vi "Drive Controller.vi"(8 "error in":errorcluster) -> ()   [LabVIEW 2025]
doc: "This VI executes continuously carrying out the current operation and responding to updates or new operation requests. It will often contain the timing or control code that is difficult to place directly in TeleOp. This VI generally opens all sensors and motors and isolates the rest of the robot code from knowing implementation details of how the operations are carried out."
uses:
  <vilib>/Rock Robotics/WPI/Framework/Completion Status.ctl
  Drive Setpoints.ctl
  Drive Operations.ctl
  bordeaux-main/Bordeaux/Types/Single Cmd Info.ctl
  <vilib>/picture/picture.llb/imagedata.ctl
  bordeaux-main/Bordeaux/Types/Trajectory Data.ctl
  bordeaux-main/Bordeaux/Types/Segment Type.ctl
  <vilib>/Rock Robotics/WPI/ThirdParty/REV Robotics/REVLib/Typedef/SPARK PID Gains.ctl
  <vilib>/Rock Robotics/WPI/ThirdParty/REV Robotics/REVLib/Typedef/SPARK Feed Forward Gains.ctl
  <vilib>/Rock Robotics/WPI/ThirdParty/REV Robotics/REVLib/Typedef/Spark MAX Idle Mode.ctl
  <vilib>/Rock Robotics/WPI/ThirdParty/REV Robotics/REVLib/Typedef/Spark MAX Control Type.ctl
  <vilib>/Rock Robotics/WPI/ThirdParty/REV Robotics/REVLib/SubVI/Public/SPARK Open Brushless.vi
  <vilib>/Rock Robotics/WPI/ThirdParty/REV Robotics/REVLib/SubVI/Public/SPARK Configure Power Current Limit.vi
  <vilib>/Rock Robotics/WPI/ThirdParty/REV Robotics/REVLib/SubVI/Public/SPARK Configure Follower Mode From Ref.vi
  <vilib>/Rock Robotics/WPI/ThirdParty/REV Robotics/REVLib/SubVI/Public/SPARK Configure Basic Idle Mode.vi
  <vilib>/Rock Robotics/WPI/ThirdParty/REV Robotics/REVLib/SubVI/Public/SPARK Configure Closed Loop Gains.vi
  <vilib>/Rock Robotics/WPI/ThirdParty/REV Robotics/REVLib/SubVI/Public/SPARK Get Encoder Status Velocity.vi
panel:
  out "Right Motors":cluster{"Sensor Velocity":dbl, dbl}(graph)={"Sensor Velocity"=-0.0, 428.5718688964844}
  out "Left Motors":cluster{dbl, "Sensor Velocity":dbl}(graph)={0.0, "Sensor Velocity"=337.14349365234375}
  in  "Feed Forward Gains":T1={"kV"=0.0022, "kS"=0.0, "kA"=0.0, "kG"=0.0, "kCos"=0.0, "kCosRatio"=0.0}
  in  "PID Gains":T2={"kP"=0.0003, "kI"=0.0, "kD"=0.0}
  in  "V Scale":dbl=1.0
  in  "Interactive Values":T3
  in  "Buttons":cluster{"Execute Cmd":bool, "Abort Cmd":bool}
  out "Command Timing":cluster{"Start Time (ms)":u32, "Iterations":i32}
  out "Status":T9
  out "Current\nCmd":string
  # "Interactive Command: You may fill in the settings for a command\nand schedule it with the Execute button. You can observe and abort\nany command while fine tuning the code for the controller."
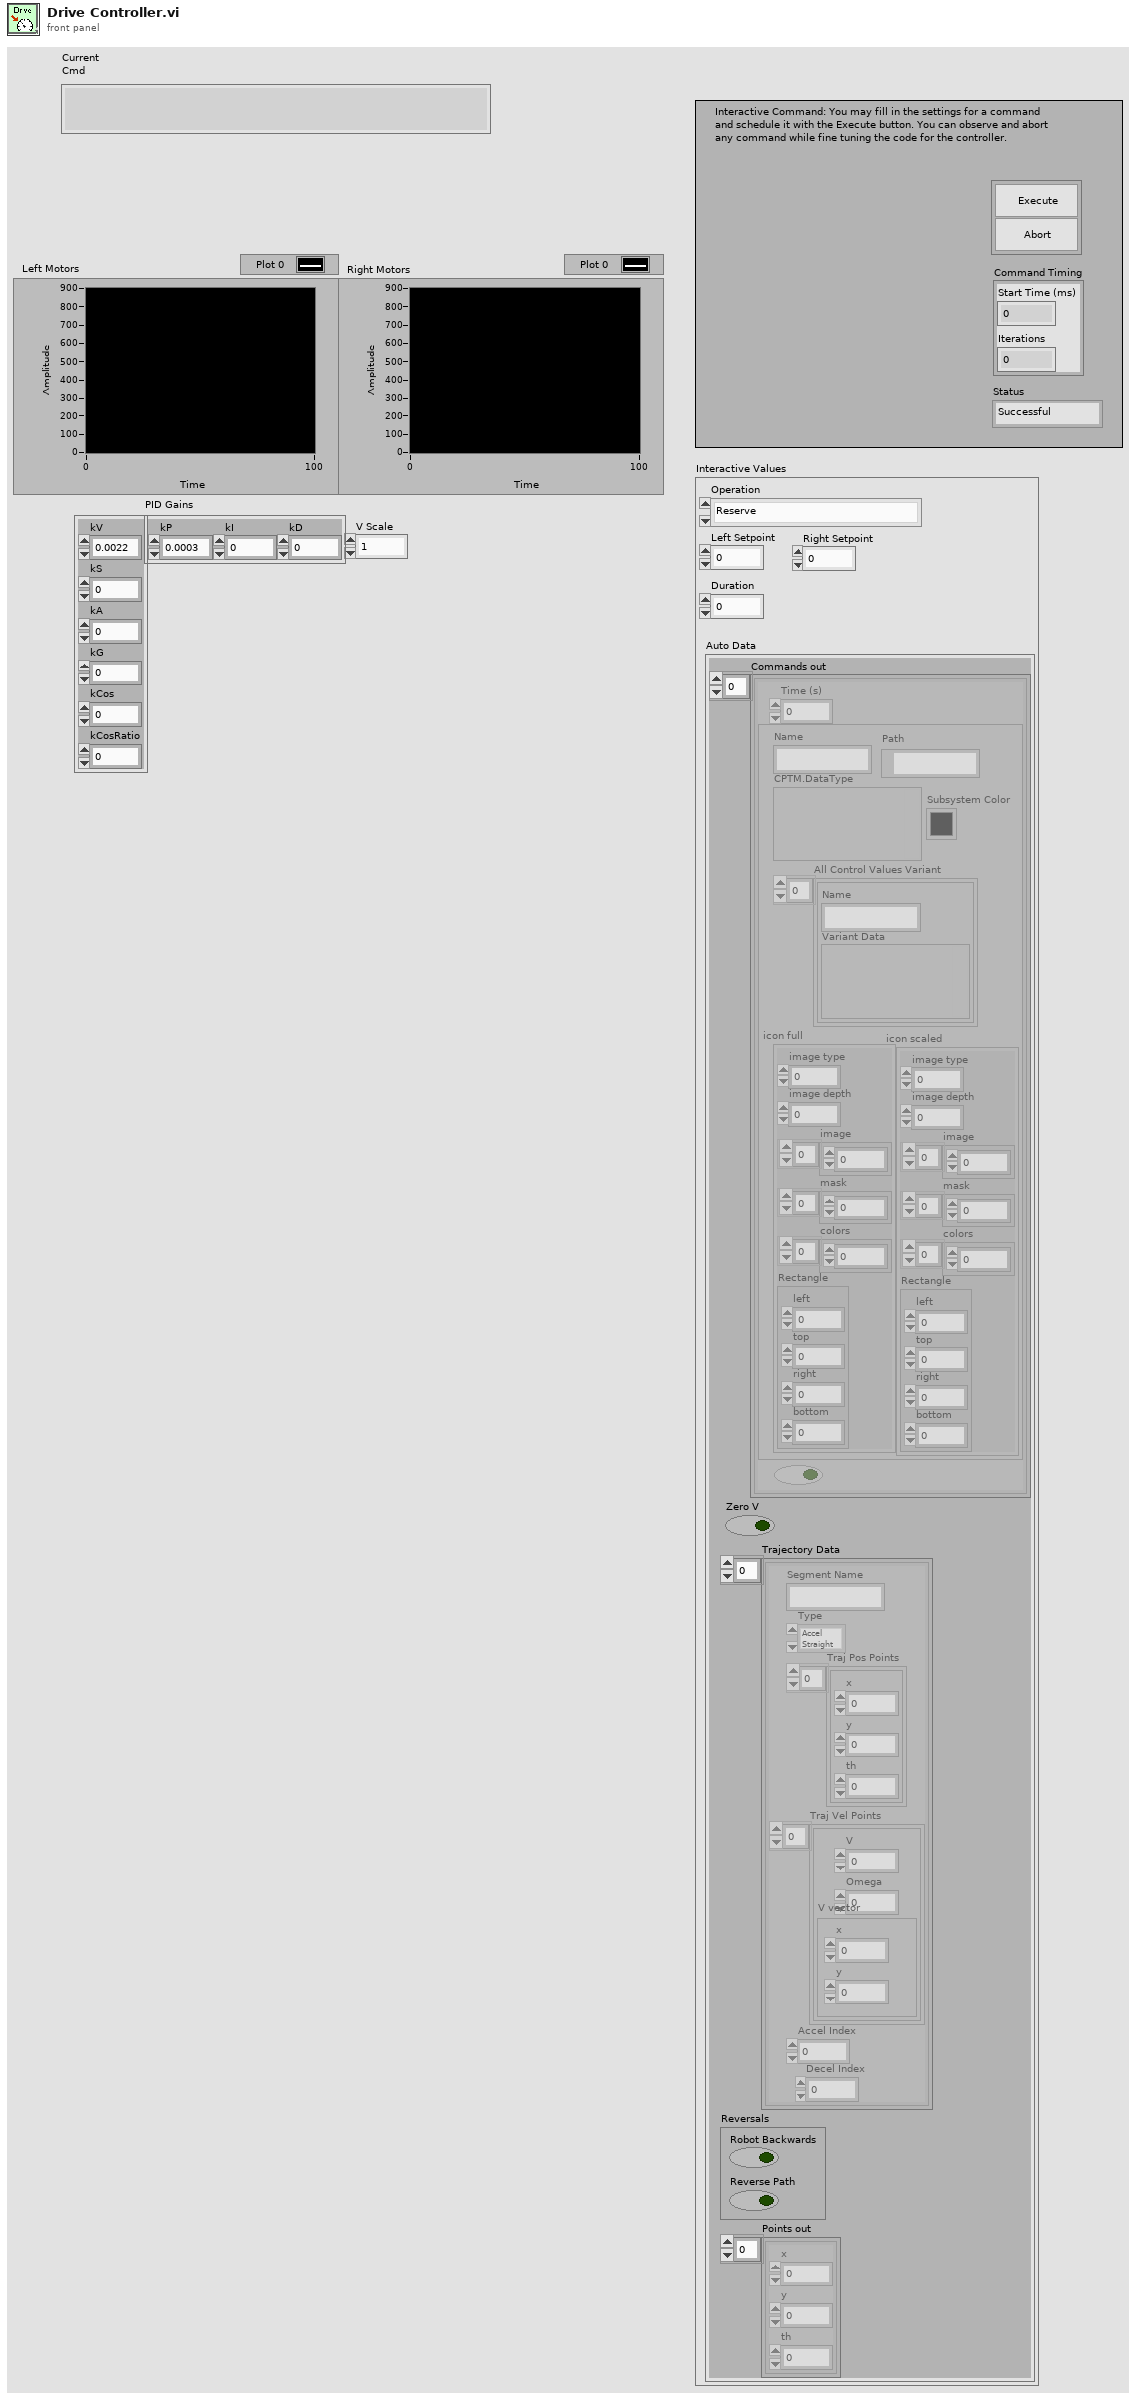
[diagram p1: front panel]
types:
  T1 = typedef "SPARK Feed Forward Gains.ctl" = cluster{"kV":dbl, "kS":dbl, "kA":dbl, "kG":dbl, "kCos":dbl, "kCosRatio":dbl}
  T2 = typedef "SPARK PID Gains.ctl" = cluster{"kP":dbl, "kI":dbl, "kD":dbl}
  T3 = typedef "Drive Setpoints.ctl" = cluster{"Operation":T4, "Left Setpoint":dbl, "Right Setpoint":dbl, "Duration":dbl, "Auto Data":cluster{"Commands out":cluster{"Time (s)":dbl, T5, bool}[], "Zero V":bool, "Trajectory Data":T7, "Reversals":cluster{"Robot Backwards":bool, "Reverse Path":bool}, "Points out":cluster{"x":dbl, "y":dbl, "th":dbl}[]}}
  T4 = typedef "Drive Operations.ctl" = enum16{"Reserve", "Read Current", "Immediate", "Drive for Time", "Play Path", "Drive for Distance"}
  T5 = typedef "Single Cmd Info.ctl" = cluster{"Name":string, "CPTM.DataType":variant, "All Control Values Variant":cluster{"Name":string, "Variant Data":variant}[], "icon full":T6, "icon scaled":T6, "Path":path, "Subsystem Color":u32}
  T6 = typedef "imagedata.ctl" = cluster{"image type":i32, "image depth":i32, "image":u8[], "mask":u8[], "colors":u32[], "Rectangle":cluster{"left":i16, "top":i16, "right":i16, "bottom":i16}}
  T7 = typedef "Trajectory Data.ctl" = cluster{"Segment Name":string, "Type":T8, "Traj Pos Points":cluster{"x":dbl, "y":dbl, "th":dbl}[], "Traj Vel Points":cluster{"V":dbl, "Omega":dbl, "V vector":cluster{"y":dbl, "x":dbl}}[], "Accel Index":i32, "Decel Index":i32}[]
  T8 = typedef "Segment Type.ctl" = enum16{"Accel Straight", "Const Straight", "Blend", "Circle", "Bezier"}
  T9 = typedef "Completion Status.ctl" = enum16{"Successful", "Aborted", "Incomplete"}
  T10 = typedef "Spark MAX Idle Mode.ctl" = enum16{"Coast", "Brake"}
  T11 = typedef "WPI_MotorControlDeviceRef.ctl" = cluster{"DeviceStatus":errorcluster, "Type":T12, "PWM":cluster{"PWM Channel":T13, "DeadBand":T14}, "CAN":cluster{"Device Number":u8, "SetOutput VI Ref":variant, "GetOutput VI Ref":variant, "Enable VI Ref":variant, "Disable VI Ref":variant, "Data":variant}, "Invert":bool, "DIO PWM":cluster{"PWM \"Enable\" Channel":T13, "DIOChannel":T15, "PWM Rate":dbl}}
  T12 = typedef "WPI_MotorControlType.ctl" = enum16{"PWM", "CAN", "DIO PWM"}
  T13 = typedef "FPGA_DIOPWMChannel.ctl" = enum8{"PWM 0", "PWM 1", "PWM 2", "PWM 3", "PWM 4", "PWM 5", "PWM 6", "PWM 7", "PWM 8", "PWM 9", "PWM MXP 0", "PWM MXP 1", "PWM MXP 2", "PWM MXP 3", "PWM MXP 4", "PWM MXP 5", "PWM MXP 6", "PWM MXP 7", "PWM MXP 8", "PWM MXP 9", "Invalid"}
  T14 = typedef "WPI_PWMDeadband.ctl" = cluster{"Name":string, "maxPositivePwm":i32, "minPositivePwm":i32, "centerPwm":i32, "maxNegativePwm":i32, "minNegativePwm":i32, "angularRange":u16}
  T15 = typedef "FPGA_DIOChannel.ctl" = enum8{"DIO 0", "DIO 1", "DIO 2", "DIO 3", "DIO 4", "DIO 5", "DIO 6", "DIO 7", "DIO 8", "DIO 9", "DIO MXP 0", "DIO MXP 1", "DIO MXP 2", "DIO MXP 3", "DIO MXP 4", "DIO MXP 5", "DIO MXP 6", "DIO MXP 7", "DIO MXP 8", "DIO MXP 9", "DIO MXP 10", "DIO MXP 11", "DIO MXP 12", "DIO MXP 13", "DIO MXP 14", "DIO MXP 15", "SPI Port CS1", "SPI Port CS2", "SPI Port CS3", "SPI Port MISO", "SPI Port MOSI", "Invalid"}
  T16 = typedef "Command Status Info.ctl" = cluster{"Name":string, "Status":T9, "notifier out":T17}
  T17 = typedef "Completion Notifier.ctl" = refnum<notifier>
  T18 = cluster{"SubSystem Data":T3, cluster{"Start Time (ms)":u32, "Iterations":i32}, cluster{"Command Info":T16, "Description":string, "Default Command":T3, "queue out":refnum<queue>, "Subsystem Name":string}}
  T19 = cluster{"Commands out":cluster{"Time (s)":dbl, T5, bool}[], "Zero V":bool, "Trajectory Data":T7, "Reversals":cluster{"Robot Backwards":bool, "Reverse Path":bool}, "Points out":cluster{"x":dbl, "y":dbl, "th":dbl}[]}
  T20 = typedef "Spark MAX Control Type.ctl" = enum16{"Percent VBus", "Voltage", "Velocity", "Position", "Smart Motion", "Current", "Smart Velocity", "MAXMotion Position", "MAXMotion Velocity"}
  T21 = cluster{"SubSystem Data":T3, cluster{"Start Time (ms)":u32, "Iterations":i32}, "Default Command Arguments":cluster{"Command Info":T16, "Description":string, "Default Command":T3, "queue out":refnum<queue>, "Subsystem Name":string}}
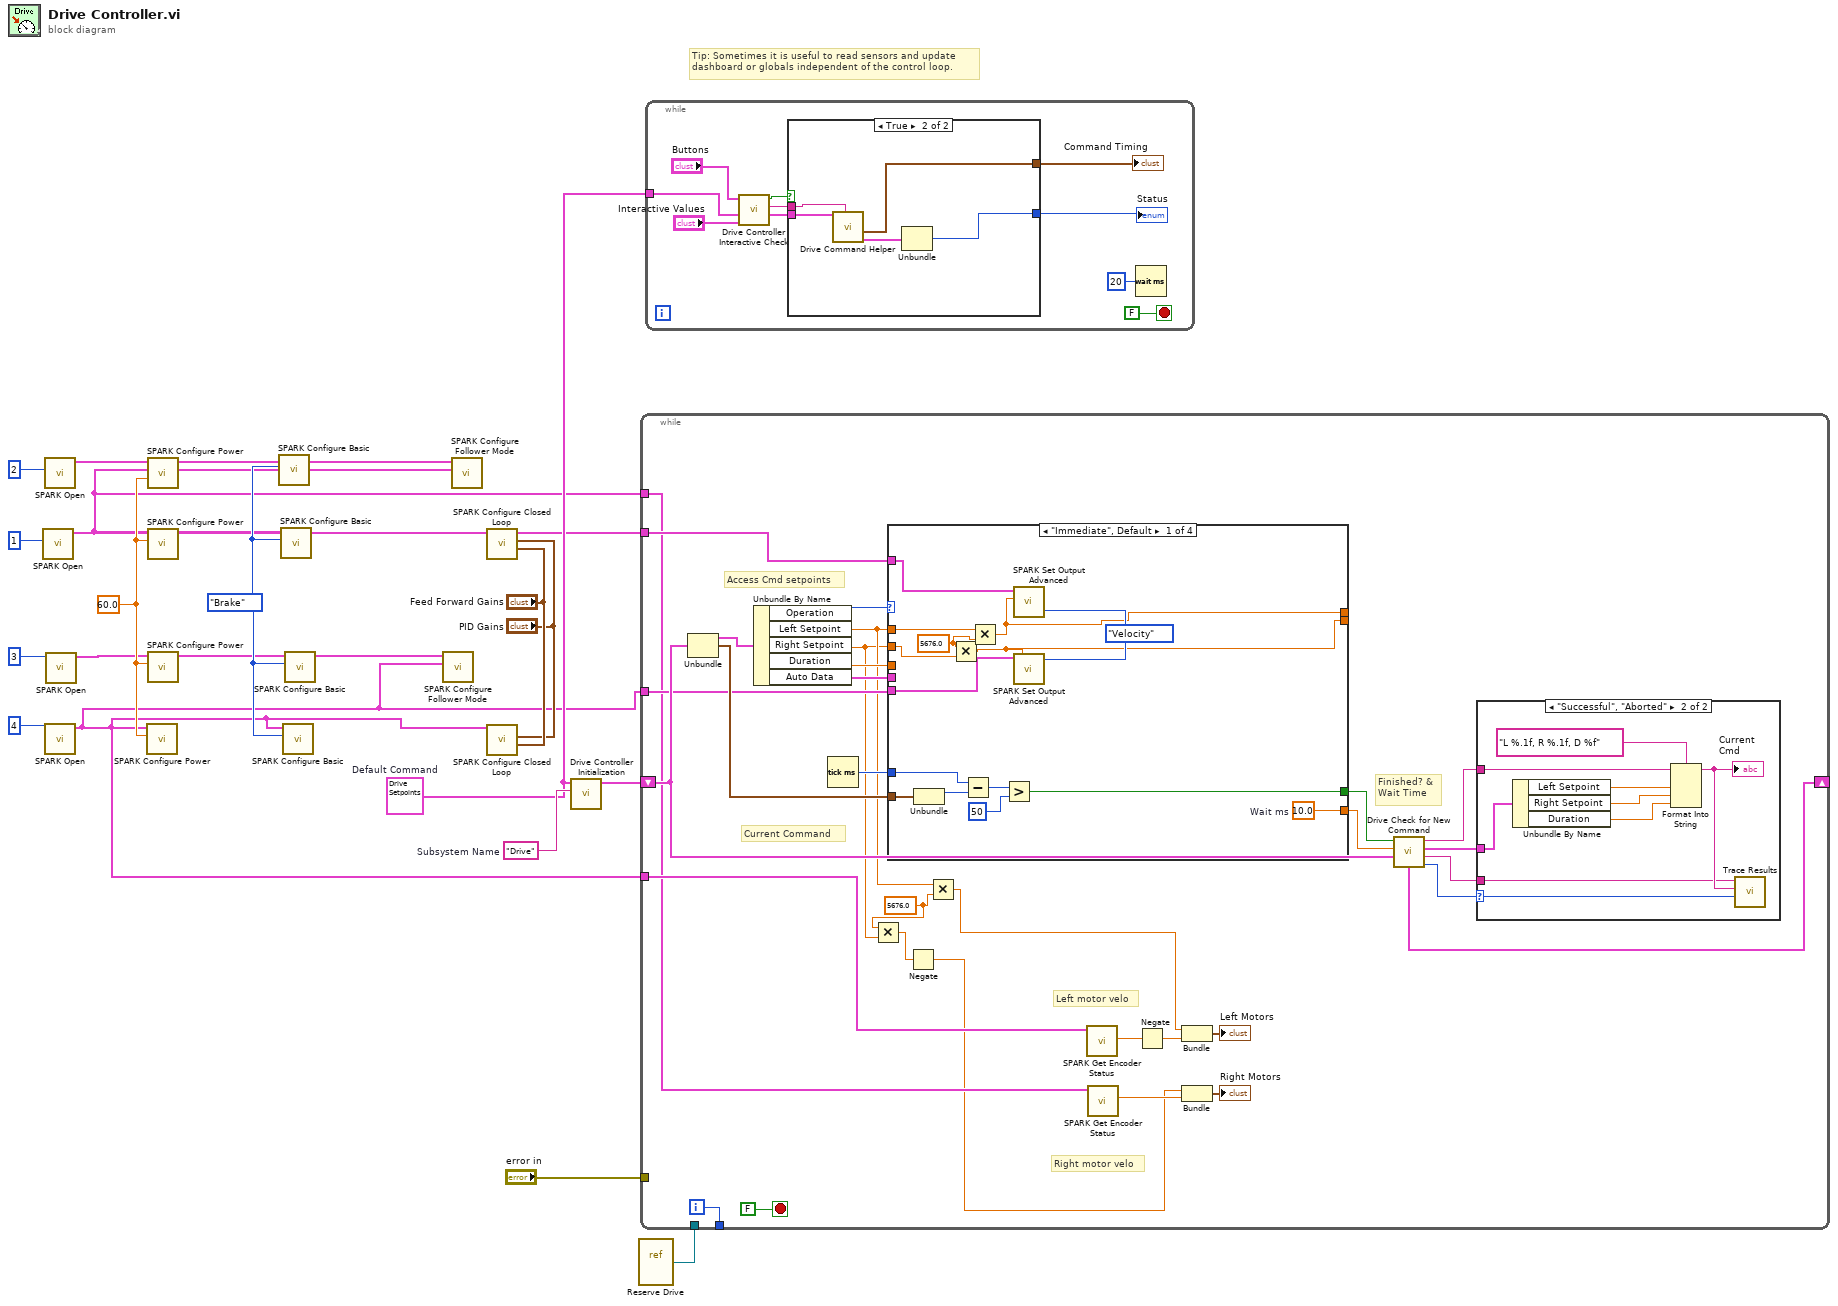
[diagram p0: block diagram]
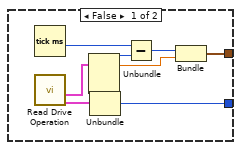
[diagram p2: hidden frame]
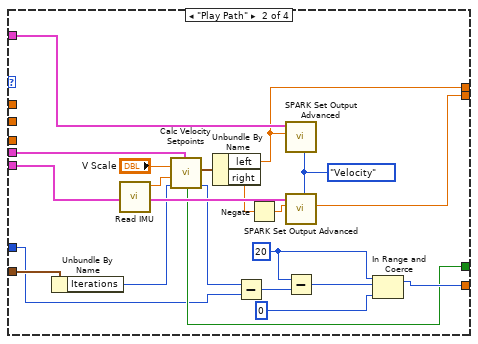
[diagram p4: hidden frame]
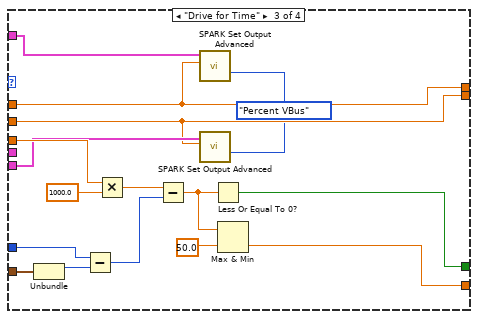
[diagram p5: hidden frame]
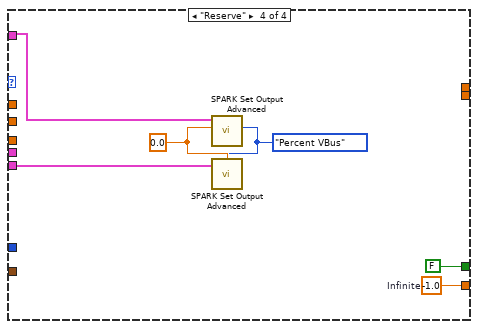
[diagram p6: hidden frame]
diagram:
  w7 = Spark_MAX_Idle_Mode."Brake" ("Idle Mode")
  w8 = 60.0 ("Primay Current Limit (80A)")
  w13 = T3 {"Operation"=enum."Reserve", "Left Setpoint"=0.0, "Right Setpoint"=0.0, "Duration"=0.0, "Auto Data"={"Commands out"=[], "Zero V"=FALSE, "Trajectory Data"=[], "Reversals"={"Robot Backwards"=FALSE, "Reverse Path"=FALSE}, "Points out"=[]}}  # Default Command
  w17 = "Drive"  # Subsystem Name
  # "Tip: Sometimes it is useful to read sensors and update\ndashboard or globals independent of the control loop."
  n1 = call-poly <vilib>:"SPARK Open.vi"("Device Number"=u8 1) -> ("MotorControlDeviceRef"=w2:T11)  [unwired: 9 in, 1 out]
  n2 = call-poly <vilib>:"SPARK Open.vi"("Device Number"=u8 2) -> ("MotorControlDeviceRef"=w3:T11)  [unwired: 9 in, 1 out]
  n3 = call-poly <vilib>:"SPARK Open.vi"("Device Number"=u8 4) -> ("MotorControlDeviceRef"=w1:T11)  [unwired: 9 in, 1 out]
  n4 = call-poly <vilib>:"SPARK Open.vi"("Device Number"=u8 3) -> ("MotorControlDeviceRef"=w4:T11)  [unwired: 9 in, 1 out]
  n5 = call-poly <vilib>:"SPARK Configure Power.vi"("Current Limit A (100)"=w8, "MotorControlDeviceRef in"=w1) -> ()  [unwired: 8 in, 2 out]
  n6 = call-poly <vilib>:"SPARK Configure Power.vi"("Current Limit A (100)"=w8, "MotorControlDeviceRef in"=w3) -> ()  [unwired: 8 in, 2 out]
  n7 = call-poly <vilib>:"SPARK Configure Power.vi"("Current Limit A (100)"=w8, "MotorControlDeviceRef in"=w2) -> ()  [unwired: 8 in, 2 out]
  n8 = call-poly <vilib>:"SPARK Configure Power.vi"("Current Limit A (100)"=w8, "MotorControlDeviceRef in"=w4) -> ()  [unwired: 8 in, 2 out]
  n9 = call-poly <vilib>:"SPARK Configure Basic.vi"("Idle Mode"=w7, "MotorControlDeviceRef in"=w3) -> ()  [unwired: 8 in, 2 out]
  n10 = call-poly <vilib>:"SPARK Configure Basic.vi"("Idle Mode"=w7, "MotorControlDeviceRef in"=w2) -> ()  [unwired: 8 in, 2 out]
  n11 = call-poly <vilib>:"SPARK Configure Basic.vi"("Idle Mode"=w7, "MotorControlDeviceRef in"=w1) -> ()  [unwired: 8 in, 2 out]
  n12 = call-poly <vilib>:"SPARK Configure Basic.vi"("Idle Mode"=w7, "MotorControlDeviceRef in"=w4) -> ()  [unwired: 8 in, 2 out]
  n13 = call-poly <vilib>:"SPARK Configure Follower Mode.vi"("Leader MotorControlDeviceRef"=w1, "MotorControlDeviceRef in"=w4) -> ()  [unwired: 8 in, 2 out]
  n14 = call-poly <vilib>:"SPARK Configure Follower Mode.vi"("Leader MotorControlDeviceRef"=w2, "MotorControlDeviceRef in"=w3) -> ()  [unwired: 8 in, 2 out]
  n15 = call-poly <vilib>:"SPARK Configure Closed Loop.vi"("Feed Forward Gains"="Feed Forward Gains", "PID Gains"="PID Gains", "MotorControlDeviceRef in"=w2) -> ()  [unwired: 7 in, 2 out]
  n16 = call-poly <vilib>:"SPARK Configure Closed Loop.vi"("Feed Forward Gains"="Feed Forward Gains", "PID Gains"="PID Gains", "MotorControlDeviceRef in"=w1) -> ()  [unwired: 7 in, 2 out]
  n17 = call "Drive Controller Initialization.vi"("Subsystem Name"=w17, "Default Command"=w13) -> ("Current Command"=w15:T18)  [unwired: 9 in]
  n18 = vi-ref "Reserve Drive.vi"() -> (w14:refnum<vi>)
  n19 = while {
    shift-right: [w41] -> _
    shift-left: w15 -> [w34]
    tunnel: [w47] -> _
    tunnel: "error in" -> [_]
    tunnel: w14 -> [_]
    tunnel: w2 -> [w33]
    tunnel: w1 -> [w32]
    tunnel: w2 -> [w29]
    tunnel: w1 -> [w30]
    i -> [w47]
    stop <- FALSE stop-if-true
    w28 = 5676.0 ("y")
    # "Left motor velo"
    # "Right motor velo"
    # "Current Command"
    # "Access Cmd setpoints"
    # "Finished? &\nWait Time"
    n20 = Unbundle(w34) -> ("SubSystem Data"=w46:T3, w35:cluster{"Start Time (ms)":u32, "Iterations":i32})  [unwired: 1 out]
    n21 = Unbundle By Name(w46) -> ("Operation"=w45:T4, "Left Setpoint"=w27:dbl, "Right Setpoint"=w24:dbl, "Duration"=w44:dbl, "Auto Data"=w31:T19)
    n22 = Tick Count (ms)() -> (millisecond timer value=w43:u32)
    n23 = Multiply(x=w28, y=w24) -> (x*y=w22:dbl)
    n24 = case shown="\"Immediate\", Default" w45 {
      tunnel: [w72 w87 w98 w114] -> w40
      tunnel: [w67 w82 w103 FALSE ("ignore previous (F)")] -> w39
      tunnel: w35 -> [w66 w92 w105 _]
      tunnel: [w59 w75 w96 _] -> _
      tunnel: [w58 w74 w94 _] -> _
      tunnel: w27 -> [w61 _ w96 _]
      tunnel: w24 -> [w62 _ w94 _]
      tunnel: w44 -> [_ _ w102 _]
      tunnel: w43 -> [w68 w76 w101 _]
      tunnel: w33 -> [w65 w86 w97 w112]
      tunnel: w32 -> [w64 w85 w95 w111]
      tunnel: w31 -> [_ w83 _ _]
      frame "Immediate", Default {
        w60 = 5676.0 ("x")
        w63 = Spark_MAX_Control_Type."Velocity" ("Control Mode")
        w72 = 10.0  # Wait ms
        n25 = Unbundle(w66) -> ("Start Time (ms)"=w69:u32)  [unwired: 1 out]
        n26 = Multiply(x=w60, y=w62) -> (x*y=w58:dbl)
        n27 = Subtract(x=w68, y=w69) -> (x-y=w70:u32)
        n28 = Multiply(x=w61, y=w60) -> (x*y=w59:dbl)
        n29 = Greater?(x=w70, y=u8 50 ("Left Motor")) -> (0:w67:bool)
        n30 = call <vilib>:"SPARK Set Output Advanced.vi"("Control Mode"=w63, "Setpoint"=w59, "MotorControlDevRef"=w65) -> ()  [unwired: 7 in, 2 out]
        n31 = call <vilib>:"SPARK Set Output Advanced.vi"("Control Mode"=w63, "Setpoint"=w58, "MotorControlDevRef"=w64) -> ()  [unwired: 7 in, 2 out]
      }
      frame "Play Path" {
        w84 = Spark_MAX_Control_Type."Velocity" ("Control Mode")
        w89 = u32 20 ("x")
        n32 = Unbundle By Name(w92) -> ("Iterations"=w80:i32)
        n33 = call "Read IMU.vi"() -> ("Heading"=w78:dbl)  [unwired: 11 in]
        n34 = call "Calc Velocity Setpoints.vi"("Autos"=w83, "Iterations"=w80, "Angle"=w78, "V Scale"="V Scale") -> ("tick count(ms)"=w81:u32, "Finished?"=w82:bool, "setpoints"=w77:cluster{"left":dbl, "right":dbl})  [unwired: 5 in]
        n35 = Unbundle By Name(w77) -> ("left"=w75:dbl, "right"=w73:dbl)
        n36 = Subtract(x=w81, y=w76) -> (x-y=w90:u32)
        n37 = Negate(x=w73) -> (-x=w74:dbl)
        n38 = call <vilib>:"SPARK Set Output Advanced.vi"("Control Mode"=w84, "Setpoint"=w75, "MotorControlDevRef"=w86) -> ()  [unwired: 7 in, 2 out]
        n39 = call <vilib>:"SPARK Set Output Advanced.vi"("Control Mode"=w84, "Setpoint"=w74, "MotorControlDevRef"=w85) -> ()  [unwired: 7 in, 2 out]
        n40 = Subtract(x=w89, y=w90) -> (x-y=w91:u32)
        n41 = In Range and Coerce(upper limit=w89, x=w91, lower limit=u32 0) -> (coerced(x)=w87:u32)  [unwired: 1 out]
      }
      frame "Drive for Time" {
        w93 = Spark_MAX_Control_Type."Percent VBus" ("Control Mode")
        n42 = Unbundle(w105) -> ("Start Time (ms)"=w104:u32)  [unwired: 1 out]
        n43 = Subtract(x=w101, y=w104) -> (x-y=w108:u32)
        n44 = Multiply(x=w102, y=1000.0) -> (x*y=w107:dbl)
        n45 = Subtract(x=w107, y=w108) -> (x-y=w100:dbl)
        n46 = call <vilib>:"SPARK Set Output Advanced.vi"("Control Mode"=w93, "Setpoint"=w96, "MotorControlDevRef"=w97) -> ()  [unwired: 7 in, 2 out]
        n47 = call <vilib>:"SPARK Set Output Advanced.vi"("Control Mode"=w93, "Setpoint"=w94, "MotorControlDevRef"=w95) -> ()  [unwired: 7 in, 2 out]
        n48 = Less Or Equal To 0?(x=w100) -> (x <= 0?=w103:bool)
        n49 = Max & Min(x=w100, y=50.0) -> (min(x,y)=w98:dbl)  [unwired: 1 out]
      }
      frame "Reserve" {
        w109 = Spark_MAX_Control_Type."Percent VBus" ("Control Mode")
        w110 = 0.0 ("Don't move motors while reserved")
        w114 = -1.0  # Infinite
        n50 = call <vilib>:"SPARK Set Output Advanced.vi"("Control Mode"=w109, "Setpoint"=w110, "MotorControlDevRef"=w112) -> ()  [unwired: 7 in, 2 out]
        n51 = call <vilib>:"SPARK Set Output Advanced.vi"("Control Mode"=w109, "Setpoint"=w110, "MotorControlDevRef"=w111) -> ()  [unwired: 7 in, 2 out]
      }
    }
    n52 = Negate(x=w22) -> (-x=w21:dbl)
    n53 = Multiply(x=w27, y=w28) -> (x*y=w20:dbl)
    n54 = call-poly <vilib>:"SPARK Get Encoder Status.vi"("MotorControlDevRef in"=w30) -> ("Sensor Velocity"=w18:dbl)  [unwired: 7 in, 3 out]
    n55 = call-poly <vilib>:"SPARK Get Encoder Status.vi"("MotorControlDevRef in"=w29) -> ("Sensor Velocity"=w23:dbl)  [unwired: 7 in, 3 out]
    n56 = Negate(x=w18) -> (-x=w19:dbl)
    n57 = Bundle(w20, w19) -> (→"Left Motors":cluster{dbl, dbl})  [unwired: 1 in]
    n58 = Bundle(w21, "Sensor Velocity"=w23) -> (→"Right Motors":cluster{dbl, "Sensor Velocity":dbl})  [unwired: 1 in]
    n59 = call "Drive Check for New Command.vi"("input cluster"=w34, "Wait time (ms)"=w40, "Finished?"=w39) -> ("Completion"=w42:T9, "Subsystem Name"=w36:string, "Current Command"=w37:T3, "Initial Trace String"=w38:string, "Next Command"=w41:T21)  [unwired: 4 in]
    n60 = case shown="\"Successful\", \"Aborted\"" w42 {
      selector: w42 -> [_ w57]
      tunnel: w38 -> [_ w52]
      tunnel: w37 -> [_ w53]
      tunnel: w36 -> [_ w49]
      frame "Incomplete", Default {
        # "Continuing current command"
      }
      frame "Successful", "Aborted" {
        # "Report and setup for next command"
        n61 = Unbundle By Name(w53) -> ("Left Setpoint"=w55:dbl, "Right Setpoint"=w56:dbl, "Duration"=w50:dbl)
        n62 = Format Into String(format string="L %.1f, R %.1f, D %f", initial string=w52, w55, w56, w50) -> (resulting string=w51:string)  [unwired: 1 in, 1 out]
        "Current\nCmd" <- w51
        n63 = call <vilib>:"Trace Results.vi"("Status of previous command"=w57, "Description"=w51, "Subsystem"=w49) -> ()  [unwired: 9 in]
      }
    }
  }
  n64 = while {
    tunnel: w13 -> [w116]
    stop <- FALSE stop-if-true
    n65 = call "Drive Controller Interactive Check.vi"("Interactive Command In"="Interactive Values", "Default Command"=w116, "Buttons"="Buttons") -> ("Interactive Command Out"=w118:T3, "Trace String"=w119:string, "Schedule"=w120:bool)  [unwired: 6 in]
    n66 = case shown="True" w120 {
      tunnel: [w129 w137] -> w121
      tunnel: [w128 w133] -> w122
      tunnel: w119 -> [_ w135]
      tunnel: w118 -> [_ w134]
      frame False {
        n67 = Tick Count (ms)() -> (millisecond timer value=w132:u32)
        n68 = call "Read Drive Operation.vi"() -> ("Command Info"=w126:T16, "SubSystem Data"=w125:T3)  [unwired: 9 in, 1 out]
        n69 = Unbundle(w125) -> ("Operation"=w130:T4, "Left Setpoint"=w127:dbl)  [unwired: 3 out]
        n70 = Unbundle(w126) -> ("Status"=w129:T9)  [unwired: 2 out]
        n71 = Subtract(x=w132, y=w130) -> (x-y=w131:u32)
        n72 = Bundle(w131, "Left Setpoint"=w127) -> (w128:cluster{u32, "Left Setpoint":dbl})  [unwired: 1 in]
      }
      frame True {
        n73 = call "Drive Command Helper.vi"("Description"=w135, "SubSystem Data"=w134) -> ("Command Info Out"=w136:T16, "Command Timing"=w133:cluster{"Start Time (ms)":u32, "Iterations":i32})  [unwired: 7 in, 1 out]
        n74 = Unbundle(w136) -> ("Status"=w137:T9)  [unwired: 2 out]
      }
    }
    "Status" <- w121
    "Command Timing" <- w122
    n75 = Wait (ms)(milliseconds to wait=u32 20) -> ()  [unwired: 1 out]
  }
